vi "FuncVI_Sub - spreadsheet data to variable.vi"(4 "delimiter (Tab)":string="\t", 6 "format string":string, 7 "CE InstanceRef":T1, 8 "error in":bool, 9 "transpose":bool, 10 "spreadsheet string":string, 11 "var name":string) -> (0 "error out":bool)   [LabVIEW 2021]
doc: "::: CalcExpress Toolkit :::\nCopyright (c) 2000-2026 Konstantin Shifershteyn. All rights reserved."
uses:
  cetypes.llb/CalcExpress Instance RefNum.ctl
  cetypes.llb/VarMan Error Code.ctl
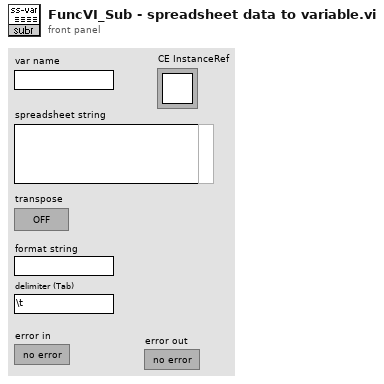
[diagram p1: front panel]
types:
  T1 = typedef "CalcExpress Instance RefNum.ctl" = refnum<k1>
  T2 = enum32{"String", "DBL Number", "identifier", "1D Array of DBL", "2D Array of DBL", "CDB Number", "1D Array of CDB", "2D Array of CDB", "1D Array of String", "2D Array of String", "Unknown data type"}
  T3 = typedef "VarMan Variable Context Handle.ctl" = i32
  T4 = typedef "VarMan Error Code.ctl" = u16
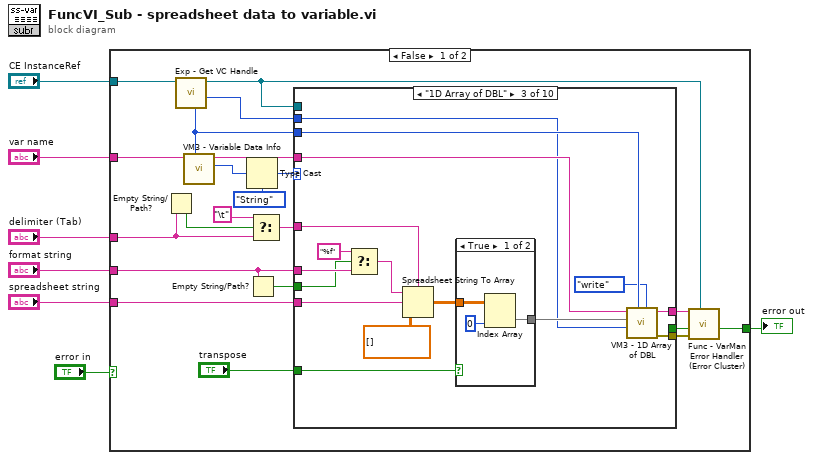
[diagram p0: block diagram]
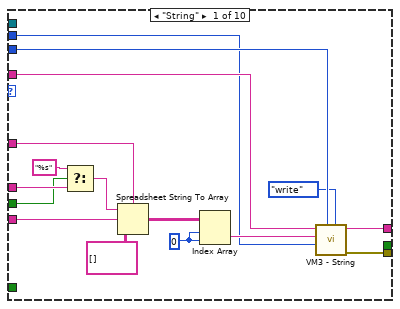
[diagram p2: hidden frame]
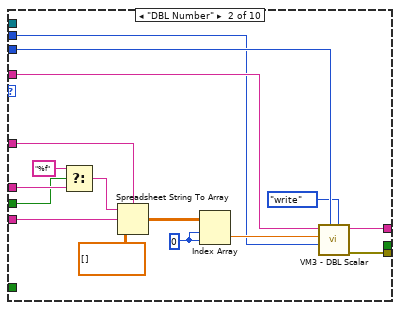
[diagram p3: hidden frame]
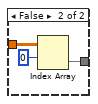
[diagram p4: hidden frame]
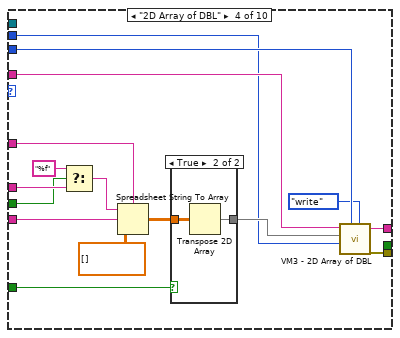
[diagram p5: hidden frame]
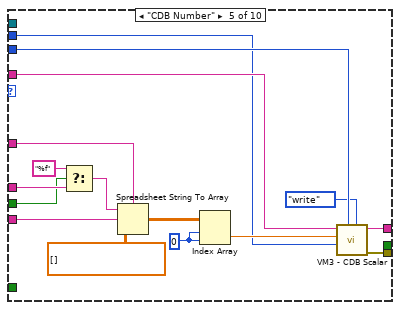
[diagram p7: hidden frame]
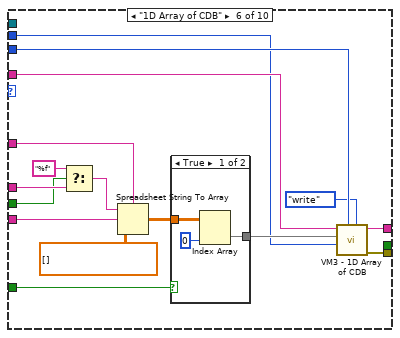
[diagram p8: hidden frame]
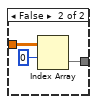
[diagram p9: hidden frame]
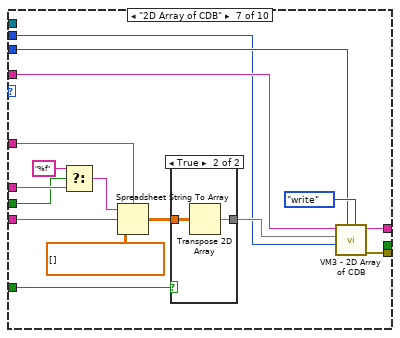
[diagram p10: hidden frame]
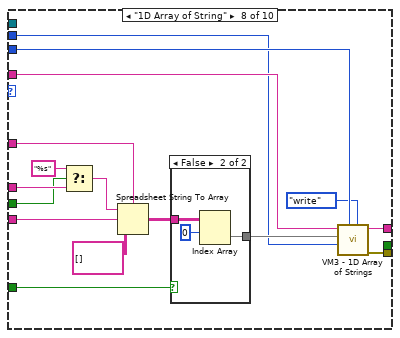
[diagram p12: hidden frame]
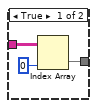
[diagram p13: hidden frame]
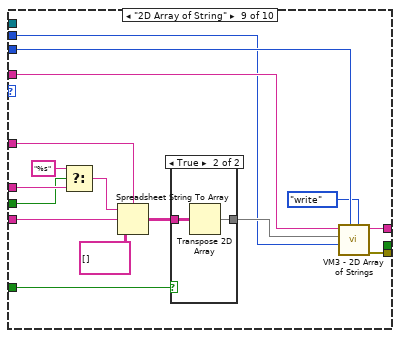
[diagram p14: hidden frame]
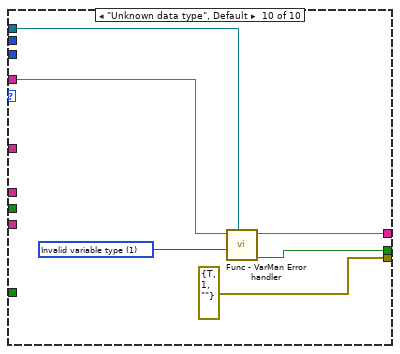
[diagram p16: hidden frame]
diagram:
  n1 = case shown="False" "error in" {
    selector: "error in" -> [_ w206]
    tunnel: [w12 w206] -> w7
    tunnel: "CE InstanceRef" -> [w19 _]
    tunnel: "var name" -> [w18 _]
    tunnel: "delimiter (Tab)" -> [w17 _]
    tunnel: "format string" -> [w16 _]
    tunnel: "spreadsheet string" -> [w15 _]
    frame False {
      n2 = Empty String/Path?(string/path=w17) -> (empty?=w21:bool)
      n3 = call "Exp - Get VC Handle.vi"("InstanceRef"=w19) -> ("writer ID"=w10:u32, "dup InstanceRef"=w9:T1, "VC Handle"=w26:T3)  [unwired: 5 in, 1 out]
      n4 = call "VM3 - Variable Data Info.vi"("VC Handle"=w26, "name_spec"=w18) -> ("var type"=w8:u32, "dup name_spec"=w23:string)  [unwired: 4 in, 4 out]
      n5 = Type Cast(type=T2."String" ("data type"), x=w8) -> (*(type *) &x=w24:T2)
      n6 = Empty String/Path?(string/path=w16) -> (empty?=w28:bool)
      n7 = Select(t="\t", s=w21, f=w17) -> (s? t:f=w20:string)
      n8 = case shown="\"1D Array of DBL\"" w24 {
        tunnel: w20 -> [w43 w59 w75 w97 w116 w132 w154 w173 w195 _]
        tunnel: w16 -> [w42 w58 w74 w96 w115 w131 w153 w172 w194 _]
        tunnel: w28 -> [w41 w57 w73 w95 w114 w130 w152 w171 w193 _]
        tunnel: w15 -> [w38 w54 w70 w92 w111 w127 w149 w168 w190 _]
        tunnel: "transpose" -> [_ _ w68 w90 _ w125 w147 w166 w188 _]
        tunnel: w23 -> [w35 w50 w63 w86 w105 w120 w142 w162 w183 w204]
        tunnel: w26 -> [w33 w49 w64 w87 w106 w122 w143 w163 w185 _]
        tunnel: [w31 w48 w65 w89 w108 w124 w145 w165 w187 w205] -> w14
        tunnel: [w30 w47 w66 w88 w107 w123 w144 w164 w186 errorcluster {"status"=TRUE, "code"=1, "source"=""} ("error out")] -> w13
        tunnel: [_ _ _ _ _ _ _ _ _ w202] -> w11
        tunnel: w10 -> [w29 w45 w62 w84 w102 w119 w140 w160 w182 _]
        tunnel: w9 -> [_ _ _ _ _ _ _ _ _ w200]
        frame "String" {
          w36 = 0
          n9 = Select(t="%s", s=w41, f=w42) -> (s? t:f=w39:string)
          n10 = Spreadsheet String To Array(delimiter (Tab)=w43, format string=w39, spreadsheet string=w38, array type (2D Dbl)=string[][] []) -> (array=w37:string[][])
          n11 = Index Array(array=w37, index (row)=w36, index (col)=w36) -> (element=w34:string)
          n12 = call "VM3 - String.vi"("cmd (read)"=enum16{"create", "destroy", "write", "read"}."write", "VC Handle"=w33, "writer ID"=w29, "value in"=w34, "name_spec"=w35) -> ("error out"=w30:errorcluster, "dup name_spec"=w31:string)  [unwired: 3 in, 2 out]
        }
        frame "DBL Number" {
          w52 = 0
          n13 = Select(t="%f", s=w57, f=w58) -> (s? t:f=w55:string)
          n14 = Spreadsheet String To Array(delimiter (Tab)=w59, format string=w55, spreadsheet string=w54, array type (2D Dbl)=dbl[][] []) -> (array=w53:dbl[][])
          n15 = Index Array(array=w53, index (row)=w52, index (col)=w52) -> (element=w51:dbl)
          n16 = call "VM3 - DBL Scalar.vi"("cmd (read)"=enum16{"create", "destroy", "write", "read"}."write", "VC Handle"=w49, "writer ID"=w45, "value in"=w51, "name_spec"=w50) -> ("error out"=w47:errorcluster, "dup name_spec"=w48:string)  [unwired: 3 in, 2 out]
        }
        frame "1D Array of DBL" {
          n17 = Select(t="%f", s=w73, f=w74) -> (s? t:f=w71:string)
          n18 = Spreadsheet String To Array(delimiter (Tab)=w75, format string=w71, spreadsheet string=w70, array type (2D Dbl)=dbl[][] []) -> (array=w69:dbl[][])
          n19 = case shown="True" w68 {
            tunnel: w69 -> [w79 w82]
            tunnel: [w77 w80] -> w67
            frame True {
              n20 = Index Array(array=w79, index (col)=0) -> (element=w77:dbl[])  [unwired: 1 in]
            }
            frame False {
              n21 = Index Array(array=w82, index (row)=0) -> (element=w80:dbl[])  [unwired: 1 in]
            }
          }
          n22 = call "VM3 - 1D Array of DBL.vi"("cmd (read)"=enum16{"create", "destroy", "write", "read"}."write", "VC Handle"=w64, "writer ID"=w62, "value in"=w67, "name_spec"=w63) -> ("error out"=w66:errorcluster, "dup name_spec"=w65:string)  [unwired: 3 in, 2 out]
        }
        frame "2D Array of DBL" {
          n23 = Select(t="%f", s=w95, f=w96) -> (s? t:f=w93:string)
          n24 = Spreadsheet String To Array(delimiter (Tab)=w97, format string=w93, spreadsheet string=w92, array type (2D Dbl)=dbl[][] []) -> (array=w91:dbl[][])
          n25 = case shown="True" w90 {
            tunnel: w91 -> [w99 w101]
            tunnel: [w99 w100] -> w85
            frame False {
            }
            frame True {
              n26 = Transpose 2D Array(2D array=w101) -> (transposed array=w100:dbl[][])
            }
          }
          n27 = call "VM3 - 2D Array of DBL.vi"("cmd (read)"=enum16{"create", "destroy", "write", "read"}."write", "VC Handle"=w87, "writer ID"=w84, "value in"=w85, "name_spec"=w86) -> ("error out"=w88:errorcluster, "dup name_spec"=w89:string)  [unwired: 3 in, 2 out]
        }
        frame "CDB Number" {
          w109 = 0
          n28 = Select(t="%f", s=w114, f=w115) -> (s? t:f=w112:string)
          n29 = Spreadsheet String To Array(delimiter (Tab)=w116, format string=w112, spreadsheet string=w111, array type (2D Dbl)=cdb[][] []) -> (array=w110:cdb[][])
          n30 = Index Array(array=w110, index (row)=w109, index (col)=w109) -> (element=w104:cdb)
          n31 = call "VM3 - CDB Scalar.vi"("cmd (read)"=enum16{"create", "destroy", "write", "read"}."write", "VC Handle"=w106, "writer ID"=w102, "value in"=w104, "name_spec"=w105) -> ("error out"=w107:errorcluster, "dup name_spec"=w108:string)  [unwired: 3 in, 2 out]
        }
        frame "1D Array of CDB" {
          n32 = Select(t="%f", s=w130, f=w131) -> (s? t:f=w128:string)
          n33 = Spreadsheet String To Array(delimiter (Tab)=w132, format string=w128, spreadsheet string=w127, array type (2D Dbl)=cdb[][] []) -> (array=w126:cdb[][])
          n34 = case shown="True" w125 {
            tunnel: w126 -> [w136 w139]
            tunnel: [w134 w137] -> w121
            frame True {
              n35 = Index Array(array=w136, index (col)=0) -> (element=w134:cdb[])  [unwired: 1 in]
            }
            frame False {
              n36 = Index Array(array=w139, index (row)=0) -> (element=w137:cdb[])  [unwired: 1 in]
            }
          }
          n37 = call "VM3 - 1D Array of CDB.vi"("cmd (read)"=enum16{"create", "destroy", "write", "read"}."write", "VC Handle"=w122, "writer ID"=w119, "value in"=w121, "name_spec"=w120) -> ("error out"=w123:errorcluster, "dup name_spec"=w124:string)  [unwired: 3 in, 2 out]
        }
        frame "2D Array of CDB" {
          n38 = Select(t="%f", s=w152, f=w153) -> (s? t:f=w150:string)
          n39 = Spreadsheet String To Array(delimiter (Tab)=w154, format string=w150, spreadsheet string=w149, array type (2D Dbl)=cdb[][] []) -> (array=w148:cdb[][])
          n40 = case shown="True" w147 {
            tunnel: w148 -> [w156 w158]
            tunnel: [w156 w157] -> w141
            frame False {
            }
            frame True {
              n41 = Transpose 2D Array(2D array=w158) -> (transposed array=w157:cdb[][])
            }
          }
          n42 = call "VM3 - 2D Array of CDB.vi"("cmd (read)"=enum16{"create", "destroy", "write", "read"}."write", "VC Handle"=w143, "writer ID"=w140, "value in"=w141, "name_spec"=w142) -> ("error out"=w144:errorcluster, "dup name_spec"=w145:string)  [unwired: 3 in, 2 out]
        }
        frame "1D Array of String" {
          n43 = Select(t="%s", s=w171, f=w172) -> (s? t:f=w169:string)
          n44 = Spreadsheet String To Array(delimiter (Tab)=w173, format string=w169, spreadsheet string=w168, array type (2D Dbl)=string[][] []) -> (array=w167:string[][])
          n45 = case shown="False" w166 {
            tunnel: w167 -> [w177 w180]
            tunnel: [w175 w178] -> w161
            frame True {
              n46 = Index Array(array=w177, index (col)=0) -> (element=w175:string[])  [unwired: 1 in]
            }
            frame False {
              n47 = Index Array(array=w180, index (row)=0) -> (element=w178:string[])  [unwired: 1 in]
            }
          }
          n48 = call "VM3 - 1D Array of Strings.vi"("cmd (read)"=enum16{"create", "destroy", "write", "read"}."write", "VC Handle"=w163, "writer ID"=w160, "value in"=w161, "name_spec"=w162) -> ("error out"=w164:errorcluster, "dup name_spec"=w165:string)  [unwired: 3 in, 2 out]
        }
        frame "2D Array of String" {
          n49 = Select(t="%s", s=w193, f=w194) -> (s? t:f=w191:string)
          n50 = Spreadsheet String To Array(delimiter (Tab)=w195, format string=w191, spreadsheet string=w190, array type (2D Dbl)=string[][] []) -> (array=w189:string[][])
          n51 = case shown="True" w188 {
            tunnel: w189 -> [w197 w199]
            tunnel: [w197 w198] -> w184
            frame False {
            }
            frame True {
              n52 = Transpose 2D Array(2D array=w199) -> (transposed array=w198:string[][])
            }
          }
          n53 = call "VM3 - 2D Array of Strings.vi"("cmd (read)"=enum16{"create", "destroy", "write", "read"}."write", "VC Handle"=w185, "writer ID"=w182, "value in"=w184, "name_spec"=w183) -> ("error out"=w186:errorcluster, "dup name_spec"=w187:string)  [unwired: 3 in, 2 out]
        }
        frame "Unknown data type", Default {
          w203 = T4 1 items=["No error", "Invalid variable type", "Variable not found", "Variable already exists", "Invalid context handle", "Input error", "Invalid data format", "No history attached", "History already attached", "Invalid history parameters", "Wrong variable name", "Wrong alias name", "Non-unique alias", "Alias not found", "No alias associated", "Alias already associated", "Wrong context name", "Non-unique context name", "Context name not found", "Invalid parameter", "Generic error", "Memory Full", "Unrecognized LV error", "Unknown error code"] ("err code")
          n54 = call "Func - VarMan Error handler.vi"("InstanceRef"=w200, "VM error code"=w203, "var name"=w204) -> ("error out"=w202:bool, "dup var name"=w205:string)  [unwired: 4 in, 1 out]
        }
      }
      n55 = call "Func - VarMan Error Handler (Error Cluster).vi"("InstanceRef"=w9, "VarMan VI error in"=w13, "error status before"=w11, "var name"=w14) -> ("FuncVI error out"=w12:bool)  [unwired: 5 in, 2 out]
    }
    frame True {
    }
  }
  "error out" <- w7
